vi "IMA Check Stop DC.vi"(0 "WFDC Notifier":refnum<notifier>, 7 "WFDC External Sync":refnum<notifier>, 11 "Error":errorcluster) -> (4 "WFDC Notifier (Dup)":refnum<notifier>, 8 "WFDC External Sync (Dup)":refnum<notifier>, 15 "Error Out":errorcluster)   [LabVIEW 2016]
uses:
  Wide Field Drift Correction/WFDC Controls/WFDC External Sync.ctl
  Wide Field Drift Correction/WFDC Controls/WFDC Cycle Pause.ctl
  Wide Field Drift Correction/WFDC Controls/WFDC Status.ctl
  Wide Field Drift Correction/WFDC Controls/WFDC Notifier Element.ctl
  Wide Field Drift Correction/WFDC Controls/WFDC Actions.ctl
  <vilib>/vision/Image Controls.llb/IMAQ Image.ctl
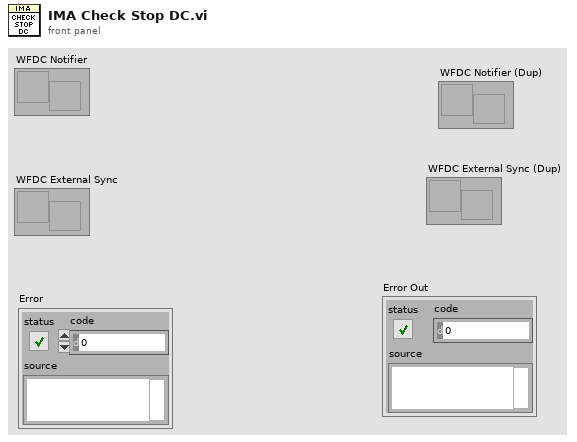
[diagram p1: front panel]
types:
  T1 = typedef "WFDC External Sync.ctl" = cluster{"Cycle Sync":T2, "Z Offset":dbl, "WFDC Status":T3}
  T2 = typedef "WFDC Cycle Pause.ctl" = enum16{"Pause Requested", "Paused", "Resume Requested", "Resumed"}
  T3 = typedef "WFDC Status.ctl" = enum16{"Idle", "Busy", "DC Active", "Error", "Canceled"}
  T4 = typedef "WFDC Notifier Element.ctl" = cluster{"WFDC Actions":T5, "Initial XYZ Positions":dbl[], "Ref Images":T6[], "Calibration (slope, inter)":dbl[], "Log Drift?":bool, "Save WF Images?":bool, "Drift Image File Ref":refnum<file>, "Drift Positions File Ref":refnum<file>, "Base Path":path, "Latest Scan Path":path, "Error":errorcluster}
  T5 = typedef "WFDC Actions.ctl" = enum16{"Error Check", "Remote Start", "Find Focus", "Pre Correct Z", "Pre Correct XY", "Setup New DC", "Setup Camera", "Get Ref Images", "Calc Calibration", "Setup Data Log", "Switch Tabs", "Get Drift / Correct Z", "Correct XY Drift", "Start Cycle", "Stop DC", "Abort Remote", "Exit Loop", "Set Error", "Generate Calibration", "Quit"}
  T6 = typedef "IMAQ Image.ctl" = refnum<image>
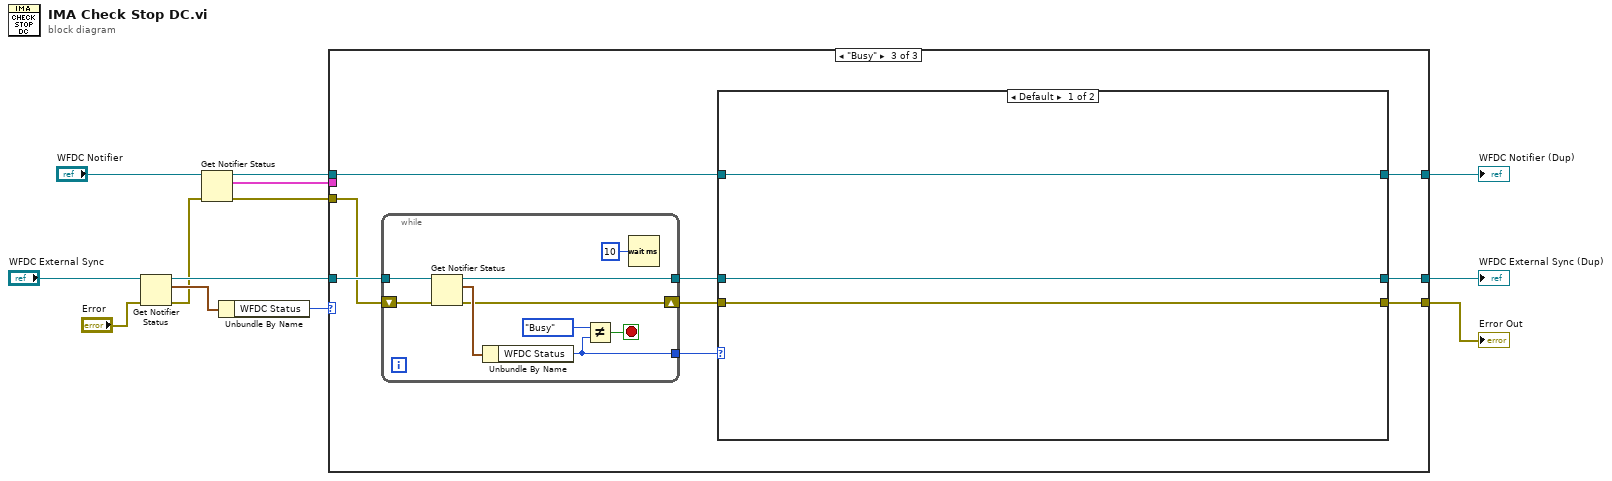
[diagram p0: block diagram]
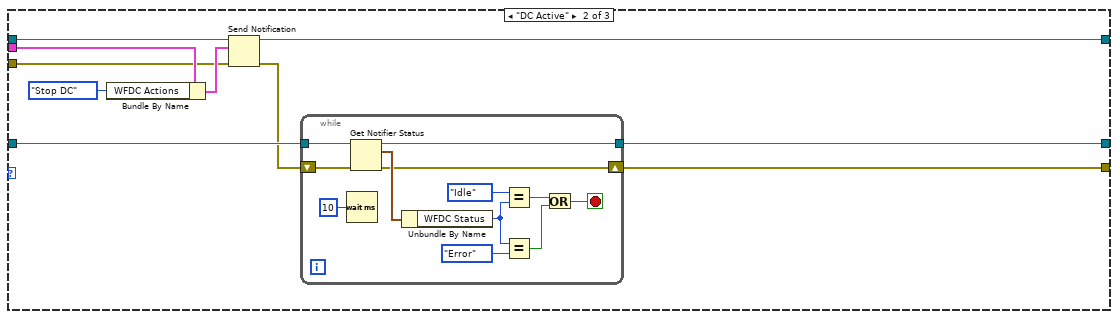
[diagram p3: hidden frame]
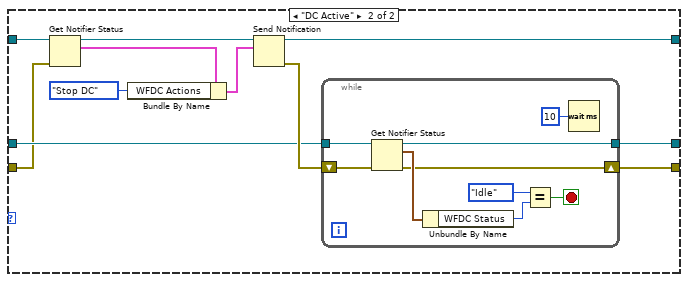
[diagram p4: hidden frame]
diagram:
  n1 = Get Notifier Status(notifier="WFDC External Sync", error in (no error)="Error") -> (notifier out=w13:refnum<notifier>, current notification=w12:T1, error out=w5:errorcluster)  [unwired: 2 out]
  n2 = Get Notifier Status(notifier="WFDC Notifier", error in (no error)=w5) -> (notifier out=w8:refnum<notifier>, current notification=w7:T4, error out=w6:errorcluster)  [unwired: 2 out]
  n3 = Unbundle By Name(w12) -> ("WFDC Status"=w11:T3)
  n4 = case shown="\"Busy\"" w11 {
    tunnel: w13 -> [w15 w22 w47]
    tunnel: w8 -> [w16 w21 w40]
    tunnel: w7 -> [_ w24 _]
    tunnel: [w16 w23 w39] -> w1
    tunnel: [w15 w18 w42] -> w2
    tunnel: w6 -> [w14 w20 w46]
    tunnel: [w14 w17 w41] -> w3
    frame Default {
    }
    frame "DC Active" {
      n5 = Bundle By Name(cluster=w24, "WFDC Actions"=WFDC_Actions."Stop DC") -> (w25:T4)
      n6 = Send Notification(notification=w25, notifier=w21, error in (no error)=w20) -> (notifier out=w23:refnum<notifier>, error out=w19:errorcluster)
      n7 = while {
        tunnel: w22 -> [w37]
        tunnel: [w35] -> w18
        shift-right: [w33] -> w17
        shift-left: w19 -> [w34]
        stop <- w27 stop-if-true
        n8 = Wait (ms)(milliseconds to wait=u32 10) -> ()  [unwired: 1 out]
        n9 = Get Notifier Status(notifier=w37, error in (no error)=w34) -> (notifier out=w35:refnum<notifier>, current notification=w38:T1, error out=w33:errorcluster)  [unwired: 2 out]
        n10 = Unbundle By Name(w38) -> ("WFDC Status"=w31:T3)
        n11 = Equal?(x=WFDC_Status."Idle", y=w31) -> (x = y?=w29:bool)
        n12 = Equal?(x=w31, y=WFDC_Status."Error") -> (x = y?=w28:bool)
        n13 = Or(x=w29, y=w28) -> (x .or. y?=w27:bool)
      }
    }
    frame "Busy" {
      n14 = while {
        tunnel: w47 -> [w78]
        tunnel: [w75] -> w44
        shift-right: [w73] -> w43
        shift-left: w46 -> [w74]
        tunnel: [w71] -> w45
        stop <- w76 stop-if-true
        n15 = Get Notifier Status(notifier=w78, error in (no error)=w74) -> (notifier out=w75:refnum<notifier>, current notification=w79:T1, error out=w73:errorcluster)  [unwired: 2 out]
        n16 = Unbundle By Name(w79) -> ("WFDC Status"=w71:T3)
        n17 = Not Equal?(x=WFDC_Status."Busy", y=w71) -> (x != y?=w76:bool)
        n18 = Wait (ms)(milliseconds to wait=u32 10) -> ()  [unwired: 1 out]
      }
      n19 = case shown="Default" w45 {
        tunnel: w44 -> [w50 w58]
        tunnel: w43 -> [w49 w51]
        tunnel: [w50 w57] -> w42
        tunnel: [w49 w56] -> w41
        tunnel: [w48 w55] -> w39
        tunnel: w40 -> [w48 w54]
        frame Default {
        }
        frame "DC Active" {
          n20 = Get Notifier Status(notifier=w54, error in (no error)=w51) -> (notifier out=w53:refnum<notifier>, current notification=w52:T4)  [unwired: 3 out]
          n21 = Bundle By Name(cluster=w52, "WFDC Actions"=WFDC_Actions."Stop DC") -> (w60:T4)
          n22 = Send Notification(notification=w60, notifier=w53) -> (notifier out=w55:refnum<notifier>, error out=w59:errorcluster)  [unwired: 1 in]
          n23 = while {
            tunnel: w58 -> [w69]
            tunnel: [w65] -> w57
            shift-right: [w63] -> w56
            shift-left: w59 -> [w64]
            stop <- w66 stop-if-true
            n24 = Get Notifier Status(notifier=w69, error in (no error)=w64) -> (notifier out=w65:refnum<notifier>, current notification=w70:T1, error out=w63:errorcluster)  [unwired: 2 out]
            n25 = Unbundle By Name(w70) -> ("WFDC Status"=w68:T3)
            n26 = Equal?(x=WFDC_Status."Idle", y=w68) -> (x = y?=w66:bool)
            n27 = Wait (ms)(milliseconds to wait=u32 10) -> ()  [unwired: 1 out]
          }
        }
      }
    }
  }
  "Error Out" <- w3
  "WFDC External Sync (Dup)" <- w2
  "WFDC Notifier (Dup)" <- w1
